vi "RemoteVI Complex Fixture All Controls.vi"(0 "Panel":refnum<vi>, 11 "error in":errorcluster) -> (4 "Controls":refnum<vi>[](array[refnum]), 15 "error out":errorcluster)   [LabVIEW 2020]
doc: "Helper of RemoteVI Complex Fixture.vi. Every control on Panel down to three levels: the top-level controls of all panes, the controls on their tab pages and in their clusters, and one level further (a cluster on a tab page). Errors of the property reads go to error out."
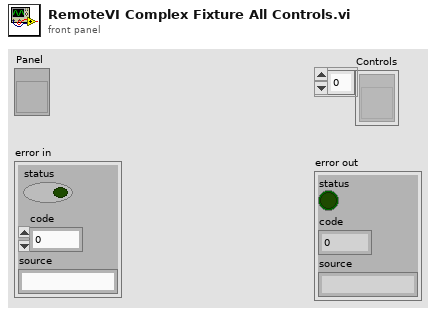
[diagram p1: front panel]
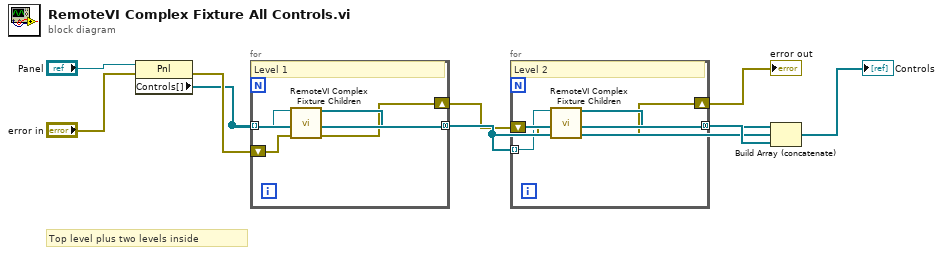
[diagram p0: block diagram]
diagram:
  # "Top level plus two levels inside"
  n1 = property class="Pnl"(reference="Panel", error in="error in") -> (error out=w4:errorcluster, "Controls[]"=w3:refnum<vi>[])  [unwired: 1 out]
  n2 = for {
    tunnel: w3 -> [w10] mode=indexing
    shift-right: [w12] -> w5
    shift-left: w4 -> [w11]
    tunnel: [w13] -> w6 mode=concatenating
    # "Level 1"
    n3 = call "RemoteVI Complex Fixture Children.vi"("Control"=w10, "error in"=w11) -> ("Children"=w13:refnum<vi>[], "error out"=w12:errorcluster)  [unwired: 12 in]
  }
  n4 = for {
    shift-right: [w16] -> w7
    shift-left: w5 -> [w15]
    tunnel: w6 -> [w14] mode=indexing
    tunnel: [w17] -> w8 mode=concatenating
    # "Level 2"
    n5 = call "RemoteVI Complex Fixture Children.vi"("Control"=w14, "error in"=w15) -> ("Children"=w17:refnum<vi>[], "error out"=w16:errorcluster)  [unwired: 12 in]
  }
  "error out" <- w7
  n6 = Build Array (concatenate)(w3, w6, w8) -> (→"Controls":refnum<vi>[])
